vi "RDC-test-Check_Error.vi"() -> ()   [LabVIEW 2020]
doc: "Checks the error of the compensated permittivity calculation, run by hand. It uses the DAK 3.5 probe values and RDC-error_check and shows the differences on the panel."
uses:
  RDC-error_metric_clust.ctl
  Reflector/RFH-common_data_format.ctl
  ff75970b-3fbb-40bd-acab-9ab774c26701.vi
  477356c8-eca1-42ff-8b0b-ffed0d9039fe.vi
  506917df-a357-4c8c-9268-b1bc48eb94a7.vi
  RDC-Reflection_Data_Computation.lvlib
  Reflector/RFH-Reflection_File_Handler.lvlib
panel:
  in  "Enable bruteforce offset":bool
  out "Avg Diff tot delta":cdb
  out "percent avg Diff tot delta":cdb
  out "RMSE Diff tot delta":cdb
  in  "C0":bool
  in  "Tau":bool
  out "Applied Tau":dbl format="%#_6e"
  out "Applied C0":dbl
  out "C0":dbl
  out "Tau":dbl format="%#_6e"
  in  "Tau Offset":dbl format="%#_6f"
  in  "C Offset":dbl format="%#_6f"
  out "RMSE Diff tot Last":cdb
  out "percent avg Diff tot last":cdb
  out "Avg Diff tot last":cdb
  out "RMSE Diff tot":cdb
  out "percent avg Diff tot":cdb
  out "Avg Diff tot":cdb
  out "Diff Imag":dbl[][](graph)
  out "percent diff imag":dbl[][](graph)
  out "percent diff real":dbl[][](graph)
  out "Array 2":string[](array[string])
  out "Diff Real":dbl[][](graph)
  out "Array":cluster{"String":string, "Error Metric":T1}[](array[cluster])
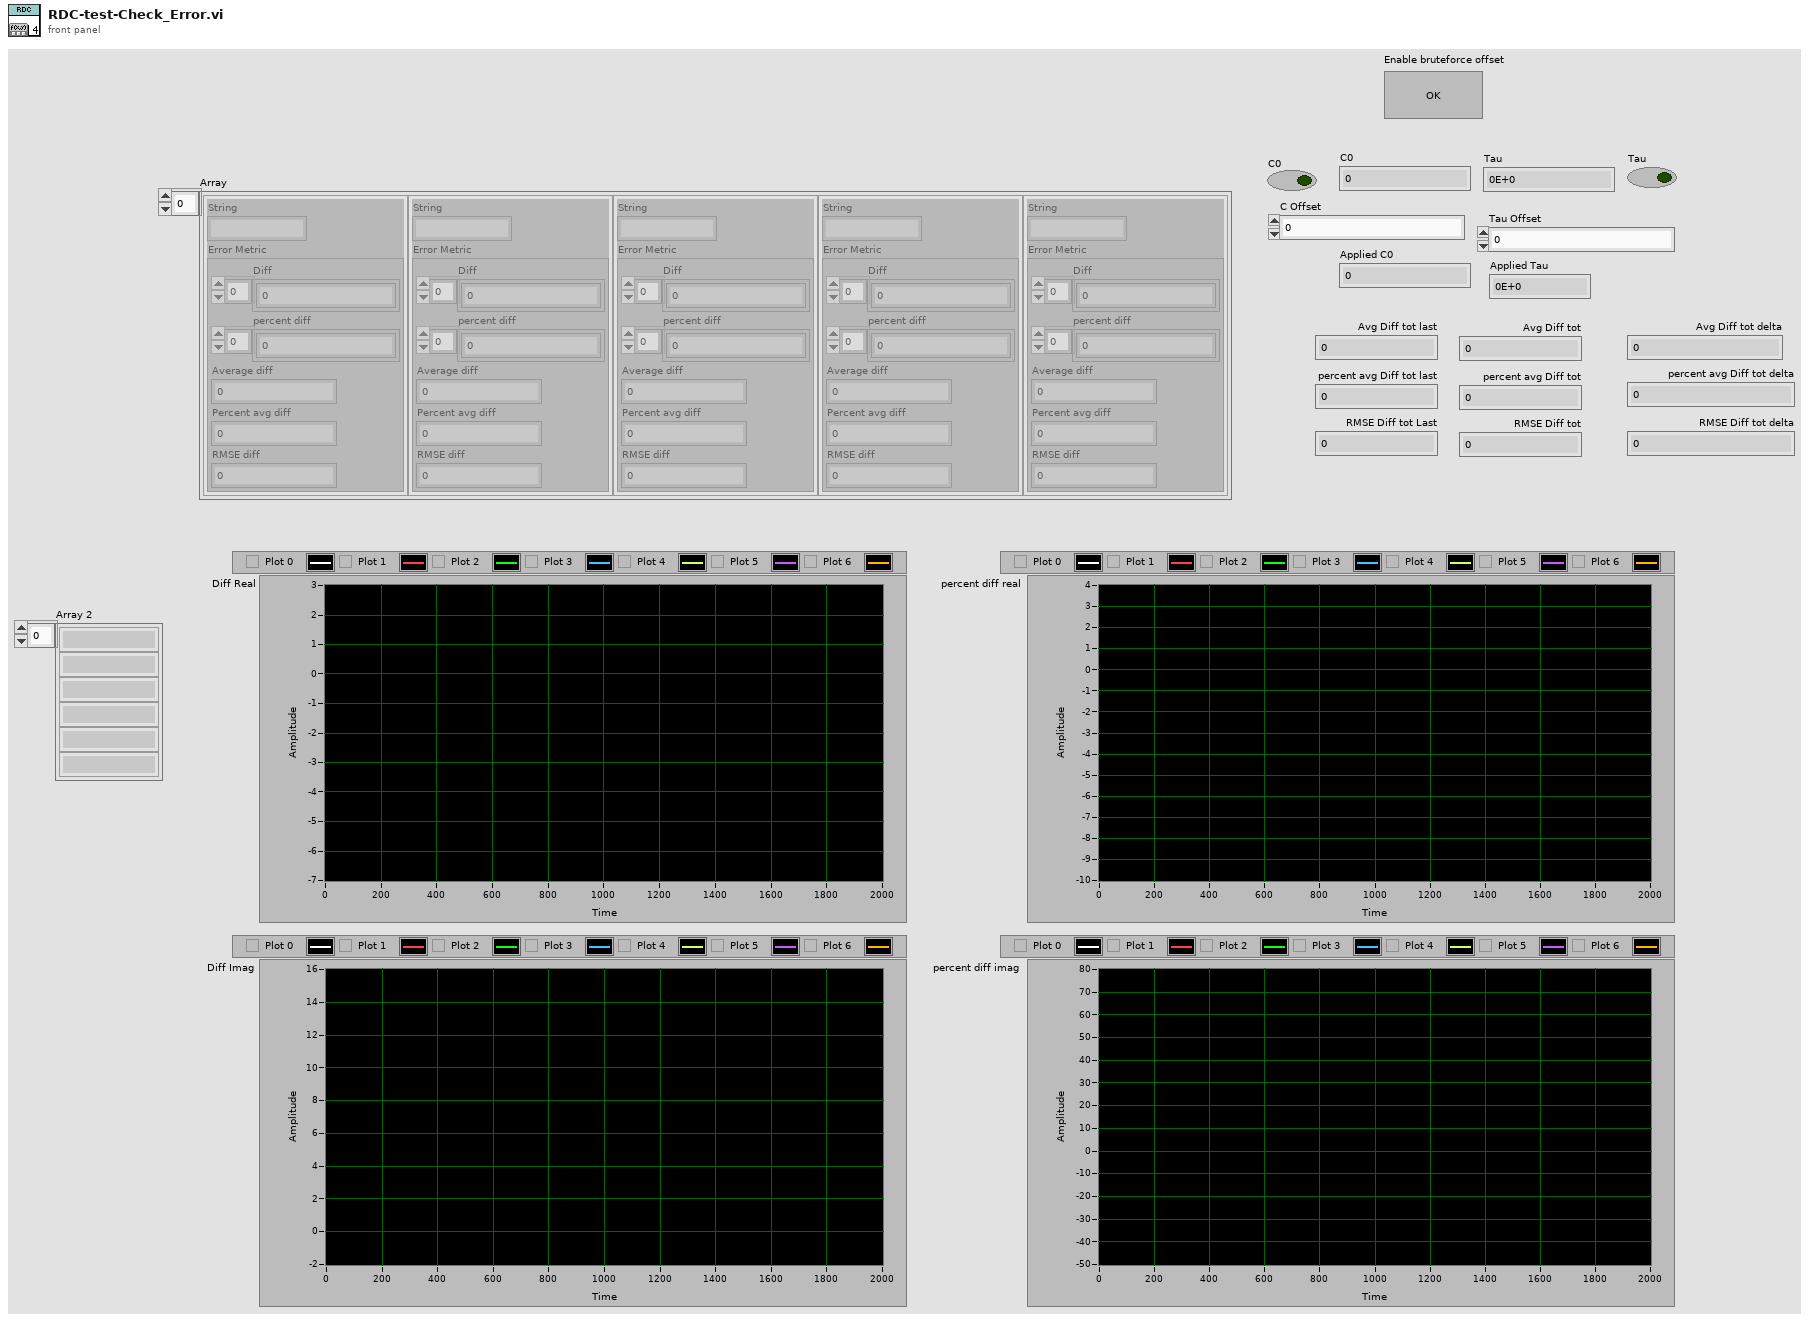
[diagram p1: front panel]
types:
  T1 = typedef "RDC-Reflection_Data_Computation.lvlib/RDC-error_metric_clust.ctl" = cluster{"Diff":cdb[], "percent diff":cdb[], "Average diff":cdb, "Percent avg diff":cdb, "RMSE diff":cdb}
  T2 = typedef "RFH-Reflection_File_Handler.lvlib/RFH-common_data_format.ctl" = cluster{"Frequency":dbl[], "Reflection'":dbl[], "Reflection''":dbl[], "Permativity'":dbl[], "Permativity''":dbl[], "Conductivity":dbl[], "Loss Tangent":dbl[], "Resistance":dbl[], "Reactance":dbl[]}
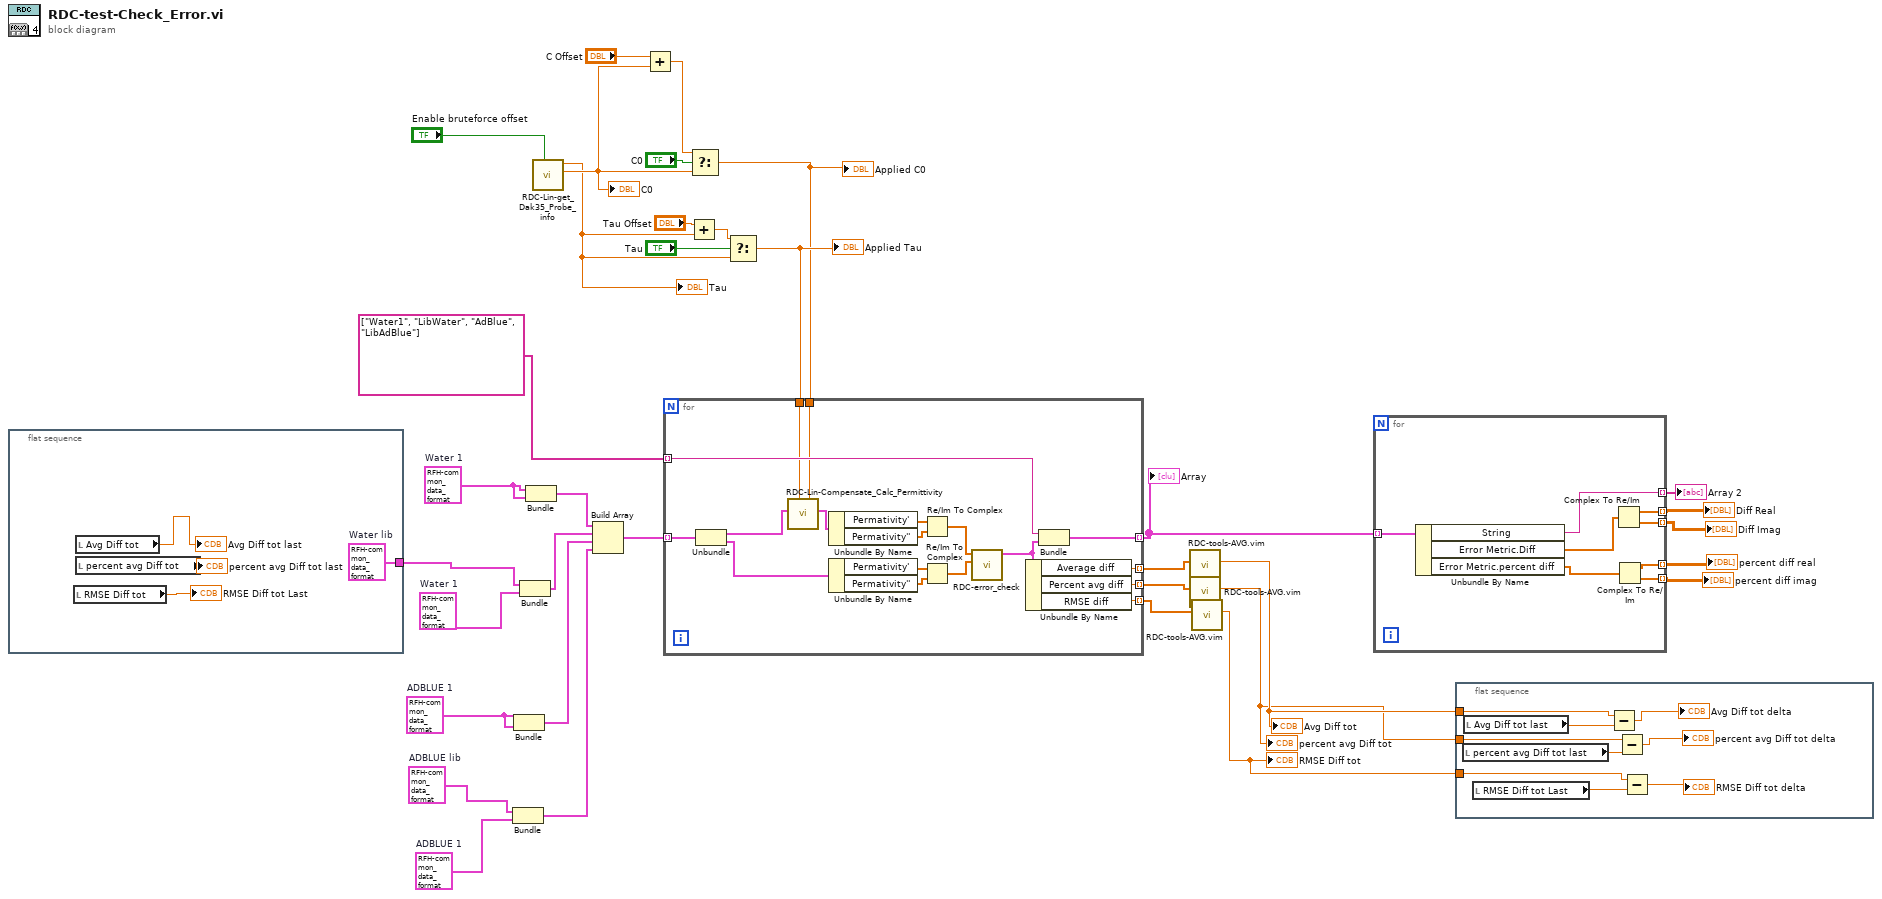
[diagram p0: block diagram]
diagram:
  w29 = T2 {"Frequency"=array[2001 elements], "Reflection'"=array[2001 elements], "Reflection''"=array[2001 elements], "Permativity'"=array[2001 elements], "Permativity''"=array[2001 elements], "Conductivity"=array[2001 elements], "Loss Tangent"=array[2001 elements], "Resistance"=[], "Reactance"=[]}  # ADBLUE 1
  w30 = T2 {"Frequency"=array[2001 elements], "Reflection'"=array[2001 elements], "Reflection''"=array[2001 elements], "Permativity'"=array[2001 elements], "Permativity''"=array[2001 elements], "Conductivity"=array[2001 elements], "Loss Tangent"=array[2001 elements], "Resistance"=[], "Reactance"=[]}  # ADBLUE lib
  w31 = T2 {"Frequency"=array[2001 elements], "Reflection'"=array[2001 elements], "Reflection''"=array[2001 elements], "Permativity'"=array[2001 elements], "Permativity''"=array[2001 elements], "Conductivity"=array[2001 elements], "Loss Tangent"=array[2001 elements], "Resistance"=[], "Reactance"=[]}  # ADBLUE 1
  w32 = T2 {"Frequency"=array[2001 elements], "Reflection'"=array[2001 elements], "Reflection''"=array[2001 elements], "Permativity'"=array[2001 elements], "Permativity''"=array[2001 elements], "Conductivity"=array[2001 elements], "Loss Tangent"=array[2001 elements], "Resistance"=[], "Reactance"=[]}  # Water 1
  w35 = T2 {"Frequency"=array[2001 elements], "Reflection'"=array[2001 elements], "Reflection''"=array[2001 elements], "Permativity'"=array[2001 elements], "Permativity''"=array[2001 elements], "Conductivity"=array[2001 elements], "Loss Tangent"=array[2001 elements], "Resistance"=[], "Reactance"=[]}  # Water 1
  n1 = flat-sequence {
    tunnel: [w39] -> w33
    frame #0 {
      w39 = T2 {"Frequency"=array[2001 elements], "Reflection'"=array[2001 elements], "Reflection''"=array[2001 elements], "Permativity'"=array[2001 elements], "Permativity''"=array[2001 elements], "Conductivity"=array[2001 elements], "Loss Tangent"=array[2001 elements], "Resistance"=[], "Reactance"=[]}  # Water lib
      n2 = local read "RMSE Diff tot"() -> (→"RMSE Diff tot Last":cdb)
      n3 = local read "Avg Diff tot"() -> (→"Avg Diff tot last":cdb)
      n4 = local read "percent avg Diff tot"() -> (→"percent avg Diff tot last":cdb)
    }
  }
  n5 = Bundle("ADBLUE lib"=w30, "ADBLUE 1"=w29) -> (w26:cluster{"ADBLUE lib":T2, "ADBLUE 1":T2})  [unwired: 1 in]
  n6 = Bundle("ADBLUE 1"=w31, "ADBLUE 1"=w31) -> (w27:cluster{"ADBLUE 1":T2, "ADBLUE 1":T2})  [unwired: 1 in]
  n7 = Bundle("Water lib"=w33, "Water 1"=w32) -> (w28:cluster{"Water lib":T2, "Water 1":T2})  [unwired: 1 in]
  n8 = Bundle("Water 1"=w35, "Water 1"=w35) -> (w34:cluster{"Water 1":T2, "Water 1":T2})  [unwired: 1 in]
  n9 = call "RDC-Lin-get_Dak35_Probe_info.vi"("Enable bruteforce offset"="Enable bruteforce offset") -> ("C0"=w12:dbl, "Tau"=w10:dbl)  [unwired: 9 in]
  "Tau" <- w10
  "C0" <- w12
  n10 = Build Array(w34, w28, w27, w26) -> (w25:cluster{"ADBLUE lib":T2, "ADBLUE 1":T2}[])
  n11 = Add(x="C Offset", y=w12) -> (x+y=w8:dbl)
  n12 = Add(x="Tau Offset", y=w10) -> (x+y=w11:dbl)
  n13 = Select(t=w8, s="C0", f=w12) -> (s? t:f=w5:dbl)
  "Applied C0" <- w5
  n14 = Select(t=w11, s="Tau", f=w10) -> (s? t:f=w6:dbl)
  "Applied Tau" <- w6
  n15 = for {
    tunnel: w25 -> [w57] mode=indexing
    tunnel: string[] ["Water1", "LibWater", "AdBlue", "LibAdBlue"] -> [w49] mode=indexing
    tunnel: [w48] -> w23 mode=indexing
    tunnel: w5 -> [w46]
    tunnel: w6 -> [w45]
    tunnel: [w42] -> w15 mode=indexing
    tunnel: [w41] -> w16 mode=indexing
    tunnel: [w40] -> w17 mode=indexing
    n16 = Unbundle(w57) -> ("ADBLUE lib"=w47:T2, "ADBLUE 1"=w52:T2)
    n17 = call "RDC-Lin-Compensate_Calc_Permittivity.vi"("C0"=w46, "Tau"=w45, "input cluster"=w47) -> ("Output cluster"=w44:T2)  [unwired: 8 in]
    n18 = Unbundle By Name(w44) -> ("Permativity'"=w56:dbl[], "Permativity''"=w55:dbl[])
    n19 = Unbundle By Name(w52) -> ("Permativity'"=w53:dbl[], "Permativity''"=w54:dbl[])
    n20 = Re/Im To Complex(1:w55, 2:w56) -> (0:w51:cdb[])
    n21 = Re/Im To Complex(1:w54, 2:w53) -> (0:w50:cdb[])
    n22 = call "RDC-error_check.vi"("Reference"=w50, "Calculated"=w51) -> ("Error Metric"=w43:T1)  [unwired: 9 in]
    n23 = Unbundle By Name(w43) -> ("Average diff"=w42:cdb, "Percent avg diff"=w41:cdb, "RMSE diff"=w40:cdb)
    n24 = Bundle("String"=w49, "Error Metric"=w43) -> (w48:cluster{"String":string, "Error Metric":T1})  [unwired: 1 in]
  }
  "Array" <- w23
  n25 = call "RDC-tools-AVG.vim"("Data Array"=w15) -> ("AVG"=w4:cdb)  [unwired: 10 in]
  "Avg Diff tot" <- w4
  n26 = call "RDC-tools-AVG.vim"("Data Array"=w16) -> ("AVG"=w3:cdb)  [unwired: 10 in]
  "percent avg Diff tot" <- w3
  n27 = call "RDC-tools-AVG.vim"("Data Array"=w17) -> ("AVG"=w2:cdb)  [unwired: 10 in]
  "RMSE Diff tot" <- w2
  n28 = for {
    tunnel: w23 -> [w65] mode=indexing
    tunnel: [w64] -> w22 mode=indexing
    tunnel: [w61] -> w20 mode=indexing
    tunnel: [w60] -> w21 mode=indexing
    tunnel: [w59] -> w19 mode=indexing
    tunnel: [w58] -> w18 mode=indexing
    n29 = Unbundle By Name(w65) -> ("String"=w64:string, "Error Metric.Diff"=w62:cdb[], "Error Metric.percent diff"=w63:cdb[])
    n30 = Complex To Re/Im(x + iy=w62) -> (x=w61:dbl[], y=w60:dbl[])
    n31 = Complex To Re/Im(x + iy=w63) -> (x=w59:dbl[], y=w58:dbl[])
  }
  "Diff Real" <- w20
  "Array 2" <- w22
  "percent diff real" <- w19
  "percent diff imag" <- w18
  "Diff Imag" <- w21
  n32 = flat-sequence {
    tunnel: w4 -> [w73]
    tunnel: w3 -> [w70]
    tunnel: w2 -> [w68]
    frame #0 {
      n33 = local read "percent avg Diff tot last"() -> (w71:cdb)
      n34 = local read "Avg Diff tot last"() -> (w74:cdb)
      n35 = local read "RMSE Diff tot Last"() -> (w69:cdb)
      n36 = Subtract(x=w73, y=w74) -> (x-y=→"Avg Diff tot delta":cdb)
      n37 = Subtract(x=w70, y=w71) -> (x-y=→"percent avg Diff tot delta":cdb)
      n38 = Subtract(x=w68, y=w69) -> (x-y=→"RMSE Diff tot delta":cdb)
    }
  }
